vi "Abort trigger.vi"(6 "Elements Available":T1, 8 "error in (no error)":errorcluster, 9 "Timed out waiting on data":bool, 10 "Logging queue element in":T3 {"Ref Dwell time (us)" format="%#.6g"; "Frame Size" items=["100X100"=100, "128X128"=128, "200X200"=200, "256X256"=256, "512X512"=512, "1024x1024"=1024, "2048x2048"=2048]; "Dwell time (us)" format="%#.6g"}, 11 "Logging queue in":T2) -> (0 "error out":errorcluster, 1 "Stop the acquisition module":bool, 2 "Logging queue metadata shift out":T3 {"Ref Dwell time (us)" format="%#.6g"; "Frame Size" items=["100X100"=100, "128X128"=128, "200X200"=200, "256X256"=256, "512X512"=512, "1024x1024"=1024, "2048x2048"=2048]; "Dwell time (us)" format="%#.6g"}, 3 "Logging queue out":T2, 4 "Force Read":bool)   [LabVIEW 2020]
uses:
  Typedefs/Logging queue element.ctl
  Typedefs/Imaging Protocols enum.ctl
  Typedefs/Frame Size.ctl
  Typedefs/Acquired points count.ctl
  Typedefs/Data queue ref.ctl
  Typedefs/FIFO elements available.ctl
  Typedefs/Read Write Enum.ctl
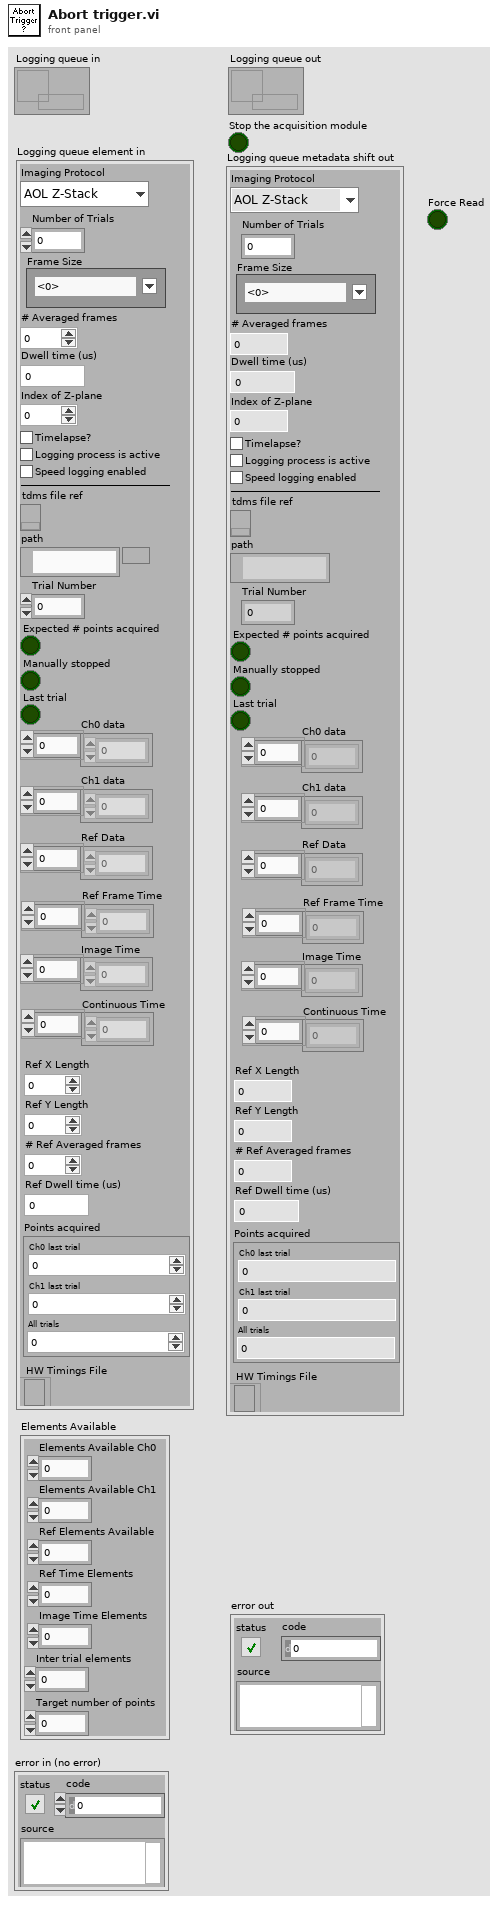
[diagram p1: front panel]
types:
  T1 = typedef "FIFO elements available.ctl" = cluster{"Elements Available Ch0":u32, "Elements Available Ch1":u32, "Ref Elements Available":u32, "Ref Time Elements":u32, "Image Time Elements":u32, "Inter trial elements":u32, "Target number of points":u64}
  T2 = typedef "Data queue ref.ctl" = refnum<queue>
  T3 = typedef "Logging queue element.ctl" = cluster{"Imaging Protocol":T4, "Number of Trials":u16, "Frame Size":T5, "# Averaged frames":u16, "Dwell time (us)":dbl, "Index of Z-plane":i32, "Timelapse?":bool, "Logging process is active":bool, "Speed logging enabled":bool, "tdms file ref":refnum<k34>, "path":path, "Trial Number":i32, "Expected # points acquired":bool, "Manually stopped":bool, "Last trial":bool, "Ch0 data":u32[], "Ch1 data":u32[], "Ref Data":u32[], "Ref Frame Time":u64[], "Image Time":u64[], "Continuous Time":u64[], "Ref X Length":u16, "Ref Y Length":u16, "# Ref Averaged frames":u16, "Ref Dwell time (us)":dbl, "Points acquired":T6, "HW Timings File":refnum<file>}
  T4 = typedef "Imaging Protocols enum.ctl" = enum16{"AOL Z-Stack", "Motor Z Stack", "Functional Acquisition", "Single Plane Acquisition", "Volume Acquisition", "Live Imaging", "Live Plane Imaging", "Live Volume Imaging"}
  T5 = typedef "Frame Size.ctl" = u16
  T6 = typedef "Acquired points count.ctl" = cluster{"Ch0 last trial":u64, "Ch1 last trial":u64, "All trials":u64}
  T7 = typedef "Read Write Enum.ctl" = enum16{"Read", "Write"}
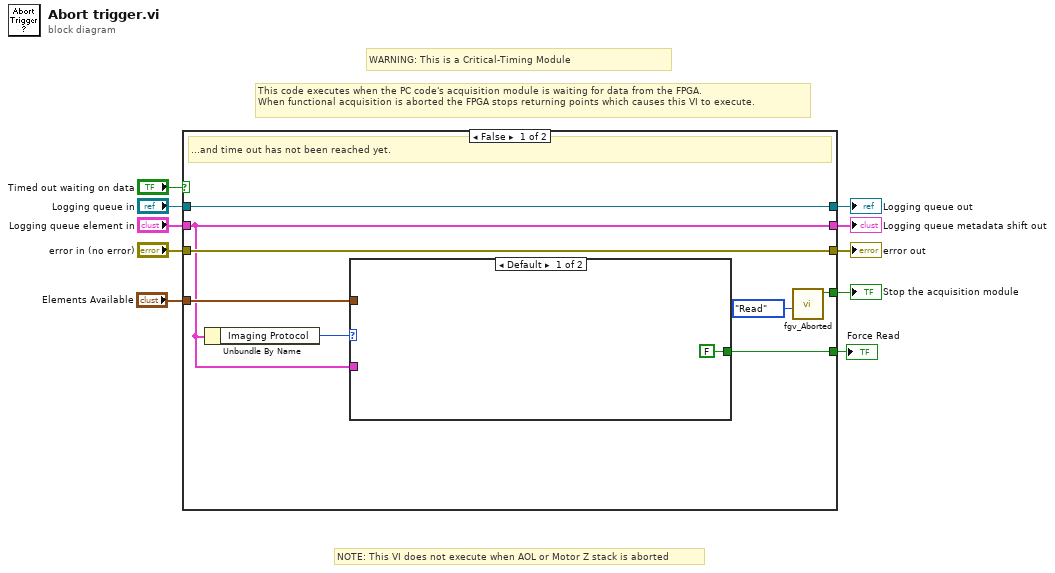
[diagram p0: block diagram]
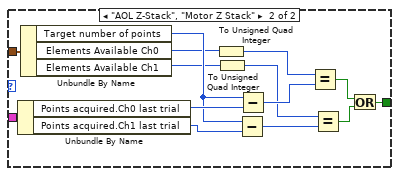
[diagram p2: hidden frame]
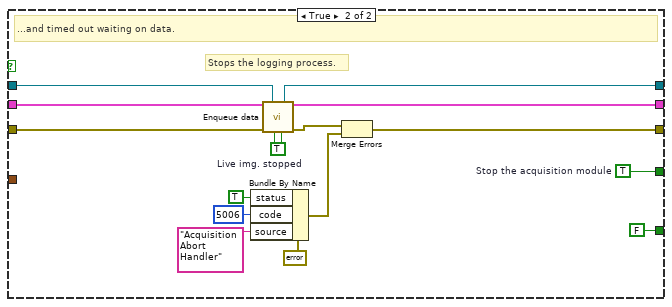
[diagram p3: hidden frame]
diagram:
  # "NOTE: This VI does not execute when AOL or Motor Z stack is aborted"
  # "WARNING: This is a Critical-Timing Module"
  # "This code executes when the PC code's acquisition module is waiting for data from the FPGA.\nWhen functional acquisition is aborted the FPGA stops returning points which causes this VI to execute."
  n1 = case shown="False" "Timed out waiting on data" {
    tunnel: [w18 w40] -> w5
    tunnel: "error in (no error)" -> [w18 w44]
    tunnel: "Logging queue in" -> [w17 w37]
    tunnel: "Logging queue element in" -> [w12 w38]
    tunnel: [w17 w36] -> w8
    tunnel: [w12 w39] -> w10
    tunnel: [w15 w35] -> w3
    tunnel: "Elements Available" -> [w14 _]
    tunnel: [w13 FALSE] -> w1
    frame False {
      # "...and time out has not been reached yet."
      n2 = Unbundle By Name(w12) -> ("Imaging Protocol"=w11:T4)
      n3 = case shown="Default" w11 {
        tunnel: w14 -> [_ w33]
        tunnel: [FALSE w21] -> w13
        tunnel: w12 -> [_ w20]
        frame Default {
        }
        frame "AOL Z-Stack", "Motor Z Stack" {
          n4 = Unbundle By Name(w20) -> ("Points acquired.Ch0 last trial"=w32:u64, "Points acquired.Ch1 last trial"=w30:u64)
          n5 = Unbundle By Name(w33) -> ("Target number of points"=w31:u64, "Elements Available Ch0"=w29:u32, "Elements Available Ch1"=w28:u32)
          n6 = To Unsigned Quad Integer(1:w29) -> (0:w27:u64)
          n7 = To Unsigned Quad Integer(1:w28) -> (0:w25:u64)
          n8 = Subtract(x=w31, y=w30) -> (x-y=w24:u64)
          n9 = Subtract(x=w31, y=w32) -> (x-y=w26:u64)
          n10 = Equal?(x=w27, y=w26) -> (x = y?=w23:bool)
          n11 = Equal?(x=w25, y=w24) -> (x = y?=w22:bool)
          n12 = Or(x=w23, y=w22) -> (x .or. y?=w21:bool)
        }
      }
      n13 = call "fgv_Aborted.vi"("Function"=Read_Write_Enum."Read") -> ("Funct Acq Aborted?"=w15:bool)  [unwired: 9 in, 1 out]
    }
    frame True {
      w35 = TRUE  # Stop the acquisition module
      w45 = TRUE  # Live img. stopped
      # "Stops the logging process."
      # "...and timed out waiting on data."
      n14 = Bundle By Name(cluster=errorcluster {"status"=FALSE, "code"=0, "source"=""} ("error out"), "status"=TRUE, "code"=5006, "source"="Acquisition Abort Handler") -> (w42:errorcluster)
      n15 = call "Enqueue data.vi"("Logging queue metadata shift in"=w38, "Logging queue in"=w37, "Error in"=w44, "Expected # points acquired"=w45, "Manually stopped"=w45) -> ("Logging queue out"=w36:T2, "Logging queue metadata shift out"=w39:T3, "error out"=w43:errorcluster)  [unwired: 8 in]
      n16 = Merge Errors(w43, w42) -> (w40:errorcluster)
    }
  }
  "Logging queue metadata shift out" <- w10
  "Logging queue out" <- w8
  "error out" <- w5
  "Stop the acquisition module" <- w3
  "Force Read" <- w1
